vi "PAQmem_FindStartStopTimeIndex.vi"(8 "error in (no error)":errorcluster, 9 "End-time":timestamp, 10 "Start-time":timestamp, 11 "PAQ-memory in":refnum<class "PAQ-memory.lvclass">) -> (0 "error out":errorcluster, 1 "Size":i32, 2 "Start":i32, 3 "PAQ-memory out":refnum<class "PAQ-memory.lvclass">, 4 "time":timestamp[](array[timestamp]))   [LabVIEW 2020, in "Sgraph_lib_V1.lvlib" / "PAQ-memory.lvclass"]
doc: "Andre Koelewijn, 2 April 2021\n\nFind the index of the start and stop time when searching for a portion of the PAQ buffer section\nAdditional to the indexes this vi also delivers the time array of the searched data portion."
uses:
  PAQ-memory.lvclass
  PAQ-memory.lvclass/PAQ-memory.ctl
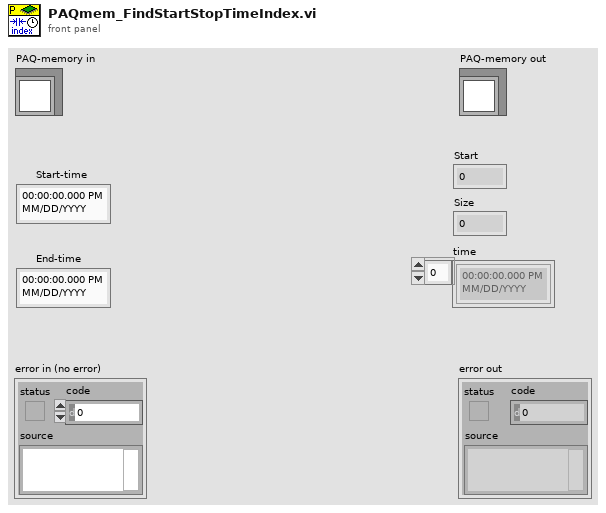
[diagram p1: front panel]
types:
  T1 = typedef "Sgraph_lib_V1.lvlib/FAMM.lvclass/typedef_PAQdata.ctl" = cluster{"TAGs":string[], "Time":refnum<data-value>, "TAGdata":cluster{"source":refnum<data-value>, "status":refnum<data-value>, "data":refnum<data-value>, "max":refnum<data-value>, "min":refnum<data-value>}[]}
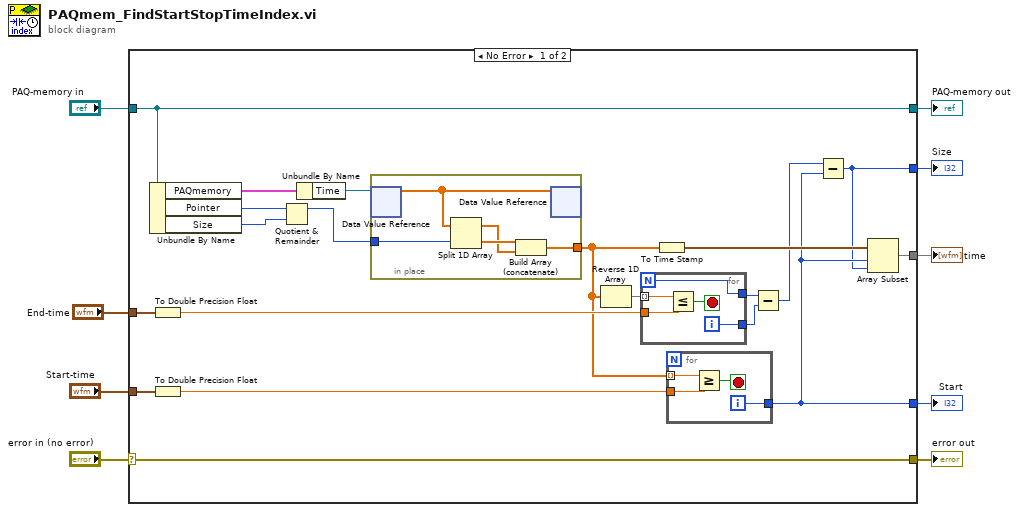
[diagram p0: block diagram]
diagram:
  n1 = case shown="No Error" "error in (no error)" {
    selector: "error in (no error)" -> [w29 w45]
    tunnel: [w29 w45] -> w8
    tunnel: [w26 w44] -> w6
    tunnel: "PAQ-memory in" -> [w26 w44]
    tunnel: [w20 _] -> w2
    tunnel: "Start-time" -> [w23 _]
    tunnel: [w16 _] -> w4
    tunnel: [w15 _] -> w3
    tunnel: "End-time" -> [w18 _]
    frame No Error {
      n2 = Unbundle By Name(w26) -> ("PAQmemory"=w28:T1, "Pointer"=w24:i32, "Size"=w19:i32)
      n3 = To Double Precision Float(number=w18) -> (double precision float=w17:dbl)
      n4 = To Double Precision Float(number=w23) -> (double precision float=w22:dbl)
      n5 = Quotient & Remainder(x=w24, y=w19) -> (x-y*floor(x/y)=w25:i32)  [unwired: 1 out]
      n6 = Unbundle By Name(w28) -> ("Time"=w27:refnum<data-value>)
      n7 = in-place {
        in-place-border: w25 -> [w42]
        in-place-border: [w39] -> w14
        n8 = in-place-dvr #1(w27) -> (w43:dbl[])  [unwired: 1 out]
        n9 = Split 1D Array(array=w43, index=w42) -> (first subarray=w40:dbl[], second subarray=w41:dbl[])
        n10 = Build Array (concatenate)(w41, w40) -> (w39:dbl[])
        n11 = in-place-dvr #1(w43) -> ()  [unwired: 2 out]
      }
      n12 = Reverse 1D Array(array=w14) -> (reversed array=w13:dbl[])
      n13 = for {
        N -> [w30]
        tunnel: w13 -> [w34] mode=indexing
        tunnel: w17 -> [w33]
        tunnel: [w31] -> w11
        tunnel: [w30] -> w12
        i -> [w31]
        stop <- w32 stop-if-true
        n14 = Less Or Equal?(x=w34, y=w33) -> (x <= y?=w32:bool)
      }
      n15 = To Time Stamp(1:w14) -> (0:w21:timestamp[])
      n16 = for {
        tunnel: w14 -> [w38] mode=indexing
        tunnel: w22 -> [w37]
        tunnel: [w35] -> w16
        i -> [w35]
        stop <- w36 stop-if-true
        n17 = Greater Or Equal?(x=w38, y=w37) -> (x >= y?=w36:bool)
      }
      n18 = Subtract(x=w12, y=w11) -> (x-y=w10:i32)
      n19 = Subtract(x=w10, y=w16) -> (x-y=w15:i32)
      n20 = Array Subset(array=w21, index=w16, length=w15) -> (w20:timestamp[])
    }
    frame Error {
    }
  }
  "error out" <- w8
  "PAQ-memory out" <- w6
  "time" <- w2
  "Start" <- w4
  "Size" <- w3
